vi "Close references.vi"(8 "references":T1) -> (0 "error out":errorcluster)   [LabVIEW 2011]
doc: "Closes references to intruments."
uses:
  Measurement References.ctl
  <vilib>/Utility/NIReport.llb/NI_report.lvclass
  <instrlib>/Agilent 3458/Agilent 3458.lvlib
  <instrlib>/Fluke 5XXX Series Multicalibrators/Fluke 5XXX Series Multicalibrators.lvlib
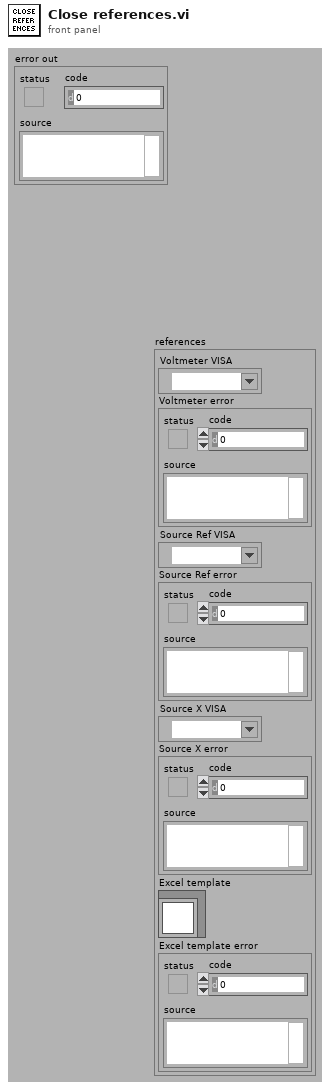
[diagram p1: front panel]
types:
  T1 = typedef "Measurement References.ctl" = cluster{"Voltmeter VISA":refnum<visa-resource-name>, "Voltmeter error":errorcluster, "Source Ref VISA":refnum<visa-resource-name>, "Source Ref error":errorcluster, "Source X VISA":refnum<visa-resource-name>, "Source X error":errorcluster, "Excel template":refnum<class "NI_report.lvclass">, "Excel template error":errorcluster}
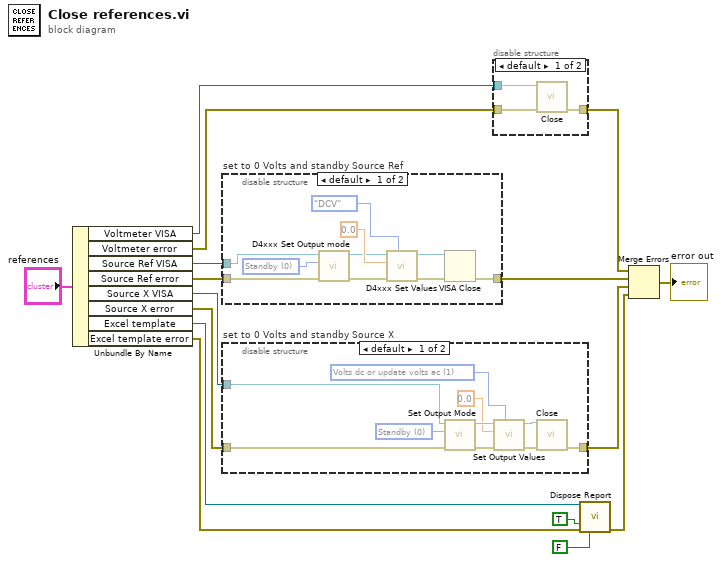
[diagram p0: block diagram]
diagram:
  n1 = Unbundle By Name("references") -> ("Voltmeter VISA"=w8:refnum<visa-resource-name>, "Voltmeter error"=w9:errorcluster, "Source Ref VISA"=w5:refnum<visa-resource-name>, "Source Ref error"=w4:errorcluster, "Source X VISA"=w7:refnum<visa-resource-name>, "Source X error"=w6:errorcluster, "Excel template"=w10:refnum<class "NI_report.lvclass">, "Excel template error"=w11:errorcluster)
  n2 = disable-structure "set to 0 Volts and standby Source Ref" shown="default" {
    disable-tunnel: [w26 w27] -> w15
    disable-tunnel: w5 -> [w20 _]
    disable-tunnel: w4 -> [w19 w27]
    frame condition #0 {
      w25 = u16 0 items=["Standby", "Operate"] ("Output mode (0:Standby)")
      n3 = call "D4xxx Set Output mode.vi"("error in"=w19, "Output mode (0:Standby)"=w25, "4808"=w20) -> ("error out"=w22:errorcluster, "Session Out"=w21:refnum<visa-resource-name>)  [unwired: 6 in]
      n4 = call "D4xxx Set Values.vi"("Function"=enum16{"DCV", "ACV", "DCI", "ACI", "R", "WBV"}."DCV", "error in"=w22, "Value"=0.0, "4xxx"=w21) -> ("error out"=w17:errorcluster, "Session Out"=w18:refnum<visa-resource-name>)  [unwired: 6 in]
      n5 = VISA Close(VISA resource name=w18, error in (no error)=w17) -> (error out=w26:errorcluster)
    }
    frame condition #1 (active) {
    }
  }
  n6 = disable-structure "set to 0 Volts and standby Source X" shown="default" {
    disable-tunnel: [w37 w38] -> w16
    disable-tunnel: w7 -> [w31 _]
    disable-tunnel: w6 -> [w30 w38]
    frame condition #0 {
      w32 = u32 1 items=["Amplitude", "Volts dc or update volts ac", "Volts ac dBm update", "Volts ac or volts dc with 0 Hz", "Volts ac in dBm", "Current dc or update current ac", "Current ac", "Update frequency", "Resistance", "Capacitance", "Temperature (Celsius)", "Temperature (Fahrenheit)", "Power dc or update power ac", "Power ac", "Dual volts dc or update dual ac", "Dual volts ac in volts", "Power ac in dBm update", "Power ac in dBm", "Dual volts ac in dBm update", "Dual volts ac in dBm"] ("Output Value(s) (0 - Amplitude)")
      w34 = u32 0 items=["Standby", "Operate"] ("Output Mode (0: Standby)")
      n7 = call <instrlib>:"Set Output Mode.vi"("error in (no error)"=w30, "Output Mode (0: Standby)"=w34, "VISA resource name"=w31) -> ("error out"=w35:errorcluster, "VISA resource name out"=w36:refnum<visa-resource-name>)  [unwired: 7 in]
      n8 = call <instrlib>:"Set Output Values.vi"("Output Value(s) (0 - Amplitude)"=w32, "error in (no error)"=w35, "Primary Value (0.0)"=0.0, "VISA resource name"=w36) -> ("error out"=w28:errorcluster, "VISA resource name out"=w29:refnum<visa-resource-name>)  [unwired: 6 in]
      n9 = call <instrlib>:"Close.vi"("VISA resource name"=w29, "error in (no error)"=w28) -> ("error out"=w37:errorcluster)  [unwired: 13 in]
    }
    frame condition #1 (active) {
    }
  }
  n10 = disable-structure shown="default" {
    disable-tunnel: [w41 w42] -> w14
    disable-tunnel: w9 -> [w40 w42]
    disable-tunnel: w8 -> [w39 _]
    frame condition #0 {
      n11 = call <instrlib>:"Close.vi"("error in (no error)"=w40, "VISA resource name"=w39) -> ("error out"=w41:errorcluster)  [unwired: 9 in]
    }
    frame condition #1 (active) {
    }
  }
  n12 = call-dynamic "Dispose Report.vi"("report in"=w10, "save changes? (F)"=TRUE, "error in (no error)"=w11, "close report? (T)"=FALSE) -> ("error out"=w2:errorcluster)  [unwired: 11 in]
  n13 = Merge Errors(w14, w15, w16, w2) -> (→"error out":errorcluster)
